vi "Edit CalcExpress Info.vi"() -> ()   [LabVIEW 2021]
doc: "::: CalcExpress Toolkit :::\nCopyright (c) 2000-2026 Konstantin Shifershteyn. All rights reserved."
panel:
  out "error out":errorcluster
  in  "CE Info VI path":path=path "../vi.lib/addons/CalcExpress/cemisc.llb/[ce] Get CE Toolkit Info.vi"
  # "Use this VI to edit the CalcExpress Toolkit version data"
  # "1. Run this VI to open the CalcExpress Information Container VI.\n2. On the Block Diagram of that VI, set the version number and release date of the CalcExpress Toolkit.\n3. Save the Information Container VI."
  # "CalcExpress Toolkit\nCopyright (c) 2000-2026 Konstantin Shifershteyn"
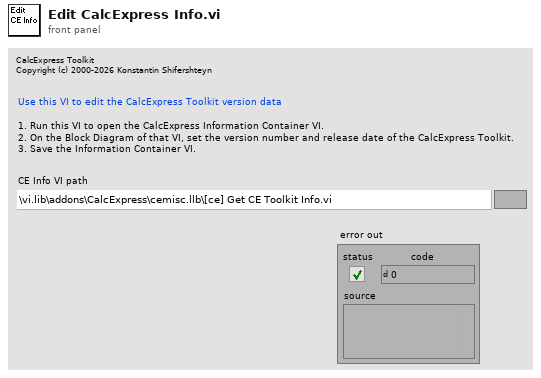
[diagram p1: front panel]
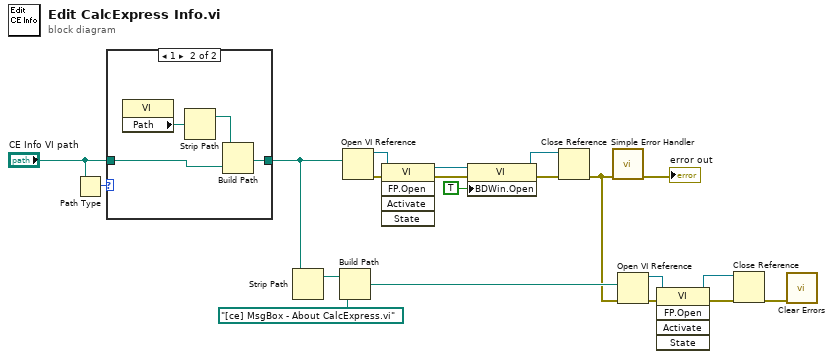
[diagram p0: block diagram]
diagram:
  n1 = Path Type(1:"CE Info VI path") -> (0:w20:i16)
  n2 = case shown="1" w20 {
    tunnel: [w21 w23] -> w3
    tunnel: "CE Info VI path" -> [w21 w24]
    frame 0, Default {
    }
    frame 1 {
      n3 = property class="VI"() -> ("Path"=w25:path)  [unwired: 2 in, 2 out]
      n4 = Strip Path(path=w25) -> (stripped path=w22:path)  [unwired: 1 out]
      n5 = Build Path(base path=w22, name or relative path=w24) -> (appended path=w23:path)
    }
  }
  n6 = Strip Path(path=w3) -> (stripped path=w10:path)  [unwired: 1 out]
  n7 = Build Path(base path=w10, name or relative path=path "[ce] MsgBox - About CalcExpress.vi") -> (appended path=w6:path)
  n8 = Open VI Reference(vi path=w3) -> (vi reference=w18:refnum<vi>, error out=w17:errorcluster)  [unwired: 5 in]
  n9 = invoke class="VI" method="FP.Open"(reference=w18, error in=w17) -> (reference out=w16:refnum<vi>, error out=w15:errorcluster)  [unwired: 3 in, 3 out]
  n10 = property class="VI"(reference=w16, error in=w15, "BDWin.Open"=TRUE ("Block Diagram Window:Open")) -> (reference out=w12:refnum<vi>, error out=w13:errorcluster)
  n11 = Close Reference(reference=w12, error in (no error)=w13) -> (error out=w1:errorcluster)
  n12 = call <vilib>:"Simple Error Handler.vi"("error in (no error)"=w1) -> ("error out"=→"error out":errorcluster)  [unwired: 4 in, 4 out]
  n13 = Open VI Reference(vi path=w6, error in (no error)=w1) -> (vi reference=w7:refnum<vi>, error out=w8:errorcluster)  [unwired: 4 in]
  n14 = invoke class="VI" method="FP.Open"(reference=w7, error in=w8) -> (reference out=w4:refnum<vi>, error out=w5:errorcluster)  [unwired: 3 in, 3 out]
  n15 = Close Reference(reference=w4, error in (no error)=w5) -> (error out=w2:errorcluster)
  n16 = call <vilib>:"Clear Errors.vi"("error in (no error)"=w2) -> ()  [unwired: 5 in, 2 out]
